vi "Read Dimensions.vi"(8 "error in":errorcluster, 11 "Array in":refnum<class "Array.lvclass">) -> (0 "error out":errorcluster, 2 "Dimensions":i32, 3 "Array out":refnum<class "Array.lvclass">)   [LabVIEW 2026, in "Array.lvclass"]
doc: "Data accessor."
uses:
  Array.lvclass
  Array.lvclass/Array.ctl
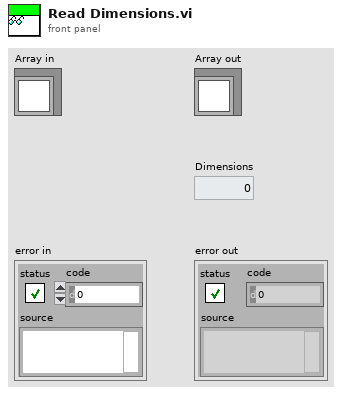
[diagram p1: front panel]
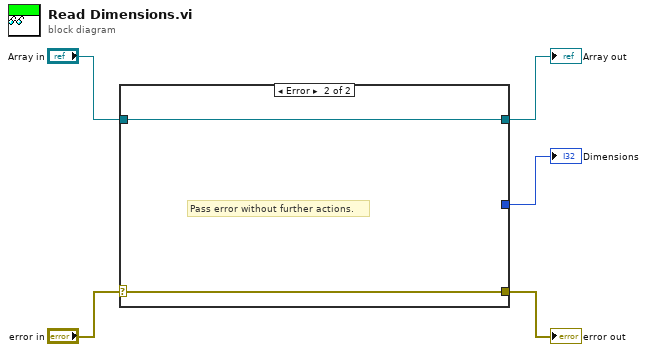
[diagram p0: block diagram]
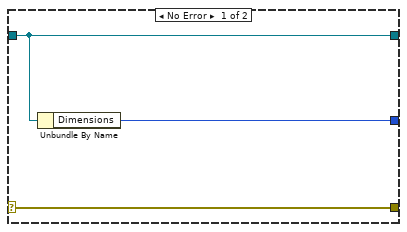
[diagram p2: hidden frame]
diagram:
  n1 = case shown="Error" "error in" {
    selector: "error in" -> [w8 w10]
    tunnel: [w8 w10] -> w4
    tunnel: [w7 w9] -> w2
    tunnel: "Array in" -> [w7 w9]
    tunnel: [w6 _] -> w1
    frame No Error {
      n2 = Unbundle By Name(w7) -> ("Dimensions"=w6:i32)
    }
    frame Error {
      # "Pass error without further actions."
    }
  }
  "error out" <- w4
  "Array out" <- w2
  "Dimensions" <- w1
